vi "CreateBodyText.vi"(9 "Body Text":T2={"Line 1 text"="", "Line 2 text"="", "Line 3 text"="", "Line 4 text"="", "Line 1 color"=0, "Line 2 color"=0, "Line 3 color"=0, "Line 4 color"=0, "Body Text Spec"={"Font"="", "Alignment"=0, "Size"=3}, "Center text vertically"=FALSE, "Capitalize Text"=FALSE} {"Body Text Spec"."Alignment" items=["left", "center", "right"]}, 10 "Path and Icon Template":T1, 11 "Icon.lvclass in":refnum<class "Icon.lvclass">) -> (1 "Body Text":picture)   [LabVIEW 2020, in "Icon Framework.lvclass"]
doc: "The incoming style information and actual text is used to actually create a picture."
uses:
  Icon Framework.lvclass
  Icon/Icon.lvclass
  Icon Framework.lvclass/Icon Framework.ctl
  resource/plugins/lv_icon.lvlib
  Controls/BodyText.ctl
  Controls/Font.ctl
  Controls/Alignment.ctl
  Controls/Graphic.ctl
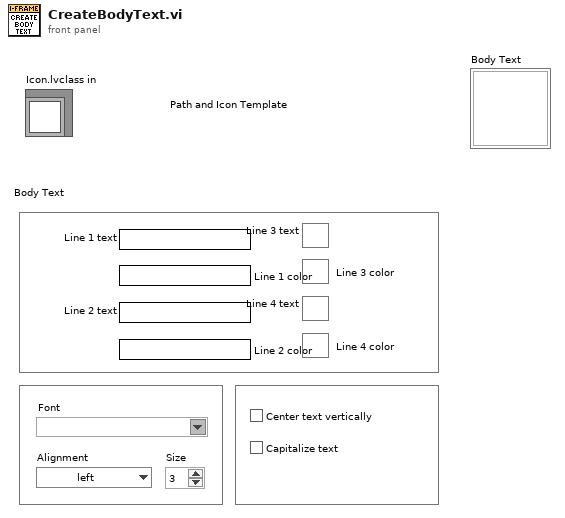
[diagram p1: front panel]
types:
  T1 = typedef "Graphic.ctl" = cluster{"Rectangle":cluster{"left":i16, "top":i16, "right":i16, "bottom":i16}, "Path":path, "Image":picture, "Filter":string, "FileName":string}
  T2 = typedef "BodyText.ctl" = cluster{"Line 1 text":string, "Line 2 text":string, "Line 3 text":string, "Line 4 text":string, "Line 1 color":u32, "Line 2 color":u32, "Line 3 color":u32, "Line 4 color":u32, "Body Text Spec":cluster{"Font":T3, "Alignment":T4, "Size":u8}, "Center text vertically":bool, "Capitalize Text":bool}
  T3 = typedef "Font.ctl" = string
  T4 = typedef "Alignment.ctl" = u16
  T5 = cluster{"horizontal":enum16{"left", "center", "right"}, "vertical":enum16{"top", "center", "bottom"}}
  T6 = cluster{"Font Name:":string, "Size":i16, "Strikeout?":bool, "Italic?":bool, "Underline?":bool, "Outline?":bool, "Shadow?":bool, "Bold?":bool}
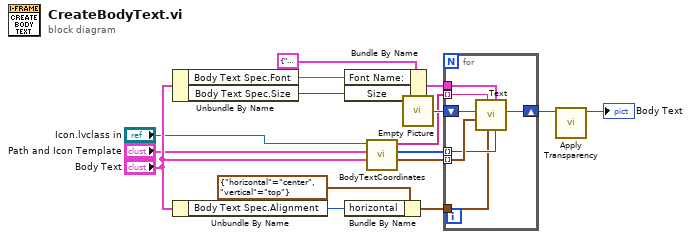
[diagram p0: block diagram]
diagram:
  n1 = Unbundle By Name("Body Text") -> ("Body Text Spec.Font"=w5:T3, "Body Text Spec.Size"=w4:u8)
  n2 = Unbundle By Name("Body Text") -> ("Body Text Spec.Alignment"=w8:T4)
  n3 = Bundle By Name(cluster=T6 {"Font Name:"="", "Size"=12, "Strikeout?"=FALSE, "Italic?"=FALSE, "Underline?"=FALSE, "Outline?"=FALSE, "Shadow?"=FALSE, "Bold?"=FALSE} ("[user-specified font]"), "Font Name:"=w5, "Size"=w4) -> (w9:T6)
  n4 = Bundle By Name(cluster=T5 {"horizontal"=enum."center", "vertical"=enum."top"} ("alignment(left, top)"), "horizontal"=w8) -> (w7:T5)
  n5 = call "BodyTextCoordinates.vi"("Body Text"="Body Text", "Path and Icon Template"="Path and Icon Template", "Icon.lvclass in"="Icon.lvclass in") -> ("Coordinates"=w15:cluster{"x":i16, "y":i16}[], "color out"=w13:u32[], "Lines out"=w14:string[])  [unwired: 5 in, 1 out]
  n6 = call "Empty Picture"() -> ("empty picture"=w16:picture)
  n7 = for {
    shift-right: [w23] -> w12
    shift-left: w16 -> [w22]
    tunnel: w14 -> [w20] mode=indexing
    tunnel: w15 -> [w21] mode=indexing
    tunnel: w13 -> [w19] mode=indexing
    tunnel: w9 -> [w18]
    tunnel: w7 -> [w17]
    n8 = call "Text.vi"("text color(black)"=w19, "[user-specified font]"=w18, "alignment(left, top)"=w17, "text"=w20, "origin"=w21, "picture"=w22) -> ("new picture"=w23:picture)  [unwired: 4 in, 1 out]
  }
  n9 = call "Apply Transparency.vi"("in"=w12) -> ("out"=→"Body Text":picture)  [unwired: 10 in]
